vi "VIH Utility - STR - Sort 1D Array of Strings w Index.vi"(6 "reverse order (F)":bool, 7 "case-sensitive sort (F)":bool, 8 "error in":errorcluster, 9 "current element index":i32, 11 "Array in":string[](array[string])) -> (0 "error out":errorcluster, 1 "new element index":i32, 2 "Index array":i32[](array[numeric]), 3 "Array out":string[](array[string]))   [LabVIEW 2014]
doc: "::: VI Helpeks :::\nCopyright (c) 2000-2026 Konstantin Shifershteyn. All rights reserved."
panel:
  # "VI Helpeks\nCopyright (c) 2012-2026 Konstantin Shifershteyn"
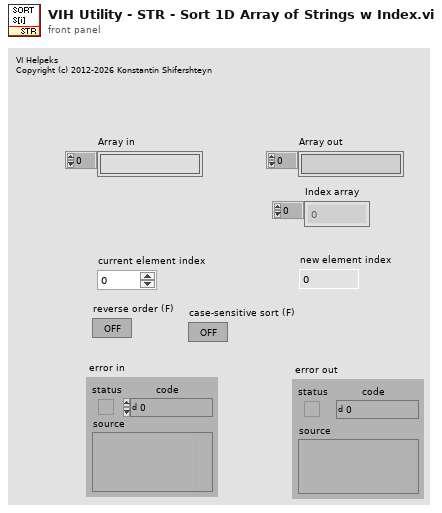
[diagram p1: front panel]
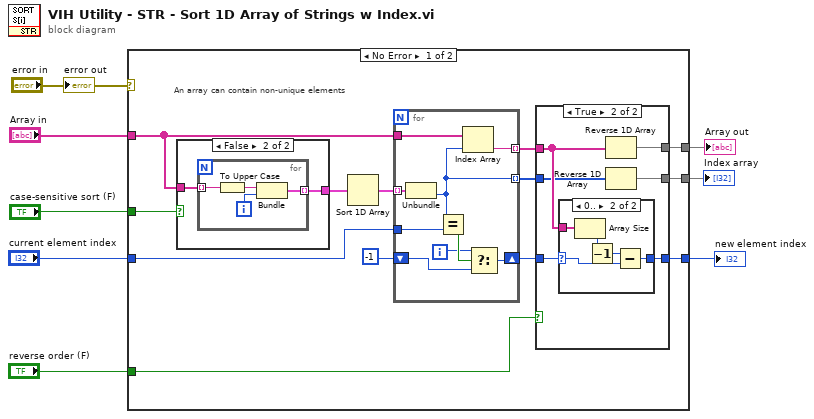
[diagram p0: block diagram]
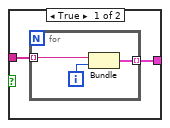
[diagram p2: hidden frame]
diagram:
  n1 = case shown="No Error" "error in" {
    tunnel: "case-sensitive sort (F)" -> [w15 _]
    tunnel: "Array in" -> [w21 w57]
    tunnel: [w19 w57] -> w6
    tunnel: "reverse order (F)" -> [w18 _]
    tunnel: [w11 w59] -> w3
    tunnel: "current element index" -> [w13 w59]
    tunnel: [w10 w58] -> w1
    frame No Error {
      # "An array can contain non-unique elements"
      n2 = case shown="False" w15 {
        tunnel: w21 -> [w23 w28]
        tunnel: [w22 w27] -> w17
        frame True {
          n3 = for {
            tunnel: w23 -> [w24] mode=indexing
            tunnel: [w25] -> w22 mode=indexing
            i -> [w26]
            n4 = Bundle("String"=w24, w26) -> (w25:cluster{"String":string, i32})  [unwired: 1 out]
          }
        }
        frame False {
          n5 = for {
            tunnel: w28 -> [w32] mode=indexing
            tunnel: [w29] -> w27 mode=indexing
            i -> [w30]
            n6 = To Upper Case(1:w32) -> (0:w31:string)
            n7 = Bundle(w31, w30) -> (w29:cluster{string, i32})  [unwired: 1 out]
          }
        }
      }
      n8 = Sort 1D Array(array=w17) -> (sorted array=w16:cluster{"String":string, i32}[])
      n9 = for {
        tunnel: w16 -> [w41] mode=indexing
        tunnel: w21 -> [w40]
        tunnel: [w39] -> w20 mode=indexing
        shift-right: [w35] -> w12
        shift-left: -1 -> [w36]
        tunnel: w13 -> [w38]
        tunnel: [w33] -> w9 mode=indexing
        i -> [w34]
        n10 = Unbundle(w41) -> (w33:i32)  [unwired: 1 out]
        n11 = Equal?(x=w33, y=w38) -> (x = y?=w37:bool)
        n12 = Index Array(array=w40, index=w33) -> (element=w39:string)
        n13 = Select(t=w34, s=w37, f=w36) -> (s? t:f=w35:i32)
      }
      n14 = case shown="True" w18 {
        tunnel: w20 -> [w44 w47]
        tunnel: [w44 w50] -> w19
        tunnel: w12 -> [w43 w49]
        tunnel: [w43 w48] -> w11
        tunnel: [w42 w46] -> w10
        tunnel: w9 -> [w42 w45]
        frame False {
        }
        frame True {
          n15 = case shown="0.." w49 {
            selector: w49 -> [w51 w55]
            tunnel: [w51 w56] -> w48
            tunnel: w47 -> [_ w52]
            frame ..-1 {
            }
            frame 0.. {
              n16 = Array Size(array=w52) -> (size(s)=w54:i32)
              n17 = Decrement(x=w54) -> (x-1=w53:i32)
              n18 = Subtract(x=w53, y=w55) -> (x-y=w56:i32)
            }
          }
          n19 = Reverse 1D Array(array=w47) -> (reversed array=w50:string[])
          n20 = Reverse 1D Array(array=w45) -> (reversed array=w46:i32[])
        }
      }
    }
    frame Error {
      n21 = for {
        tunnel: [w60] -> w58 mode=indexing
        tunnel: w57 -> [_] mode=indexing
        i -> [w60]
      }
    }
  }
  "Array out" <- w6
  "new element index" <- w3
  "Index array" <- w1
  "error out" <- "error in"
